vi "Write_Single_Impedance_Meas.vi"(0 "Meta-Data Array":dbl[](array[numeric])=[1.0], 3 "Mean Signal\nImpedance cluster":T3, 4 "Current":waveform(dbl)[](array[waveform]), 5 "Run Impedances array":dbl[][](array[numeric]), 6 "Voltage":waveform(dbl)[](array[waveform]), 7 "Compensation and Gain":T1={"Rg_Vmon"=5000.0, "Rg_Imon"=5000.0, "ESL_Cal"=2.5e-07, "ESR_Cal"=0.0, "Cp_Cal"=0.0, "Rp_Cal"=0.0, "Use Open/Short\nCompensation"=FALSE, "R_Shunt"=10000.0, "RLoad"=1000000000.0, "RLoad_Meas"=1000000000.0} {"RLoad_Meas" format="%#_6p"; "RLoad" format="%#_6p"}, 8 "Test Params Cluster":T2={"Test Freq. (Hz)"=0.0, "Output Signal Amplitude\nVolts Pk"=0.0, "Sampling Time (s)"=0.0, "Sampling Rate (Hz)"=0.0, "Output Channel"="Dev2/ao0", "Current Channel"="Dev2/ai0", "Voltage Channel"="Dev2/ai0", "Trigger Channel"="/Dev2/ao/StartTrigger", "Number of runs"=5}, 9 "Experiment Title":string="Experiment Title", 10 "File Name String":string="Test", 11 "Path":path=path "C:/Users/MPI/Documents/Test Saving Data") -> ()   [LabVIEW 2022 SP3]
panel:
  out "TDMS path":path=path "C:/Users/MPI/Documents/Test Saving Data/2022_01_06_23_07_06_Test.tdms"
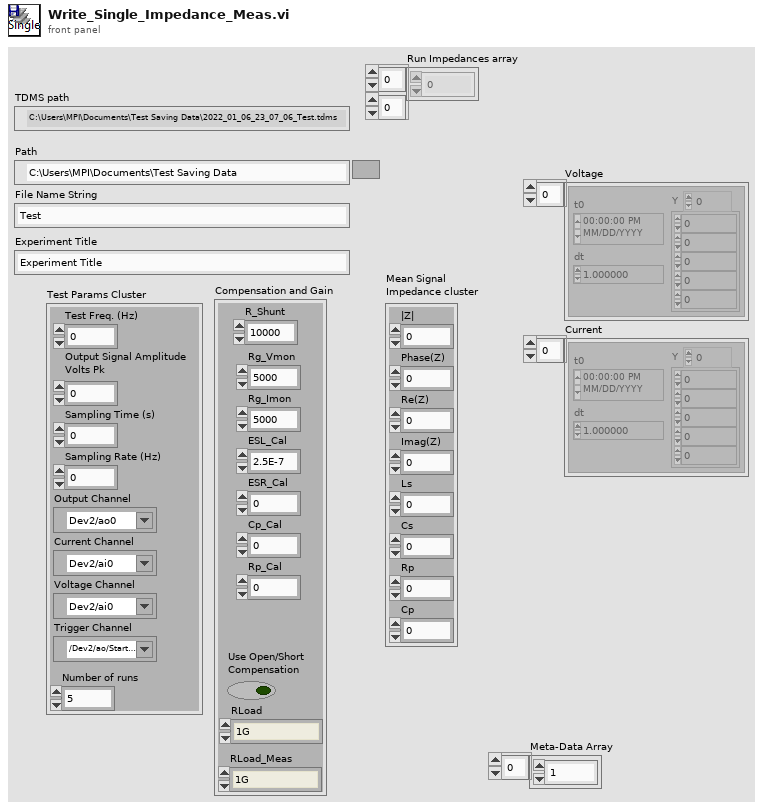
[diagram p1: front panel]
types:
  T1 = cluster{"Rg_Vmon":dbl, "Rg_Imon":dbl, "ESL_Cal":dbl, "ESR_Cal":dbl, "Cp_Cal":dbl, "Rp_Cal":dbl, "Use Open/Short\nCompensation":bool, "R_Shunt":dbl, "RLoad":dbl, "RLoad_Meas":dbl}
  T2 = cluster{"Test Freq. (Hz)":dbl, "Output Signal Amplitude\nVolts Pk":dbl, "Sampling Time (s)":dbl, "Sampling Rate (Hz)":dbl, "Output Channel":tag, "Current Channel":tag, "Voltage Channel":tag, "Trigger Channel":tag, "Number of runs":i32}
  T3 = cluster{"|Z|":dbl, "Phase(Z)":dbl, "Re(Z)":dbl, "Imag(Z)":dbl, "Ls":dbl, "Cs":dbl, "Rp":dbl, "Cp":dbl}
  T4 = enum16{"open", "open or create", "create or replace", "create", "open (read-only)"}
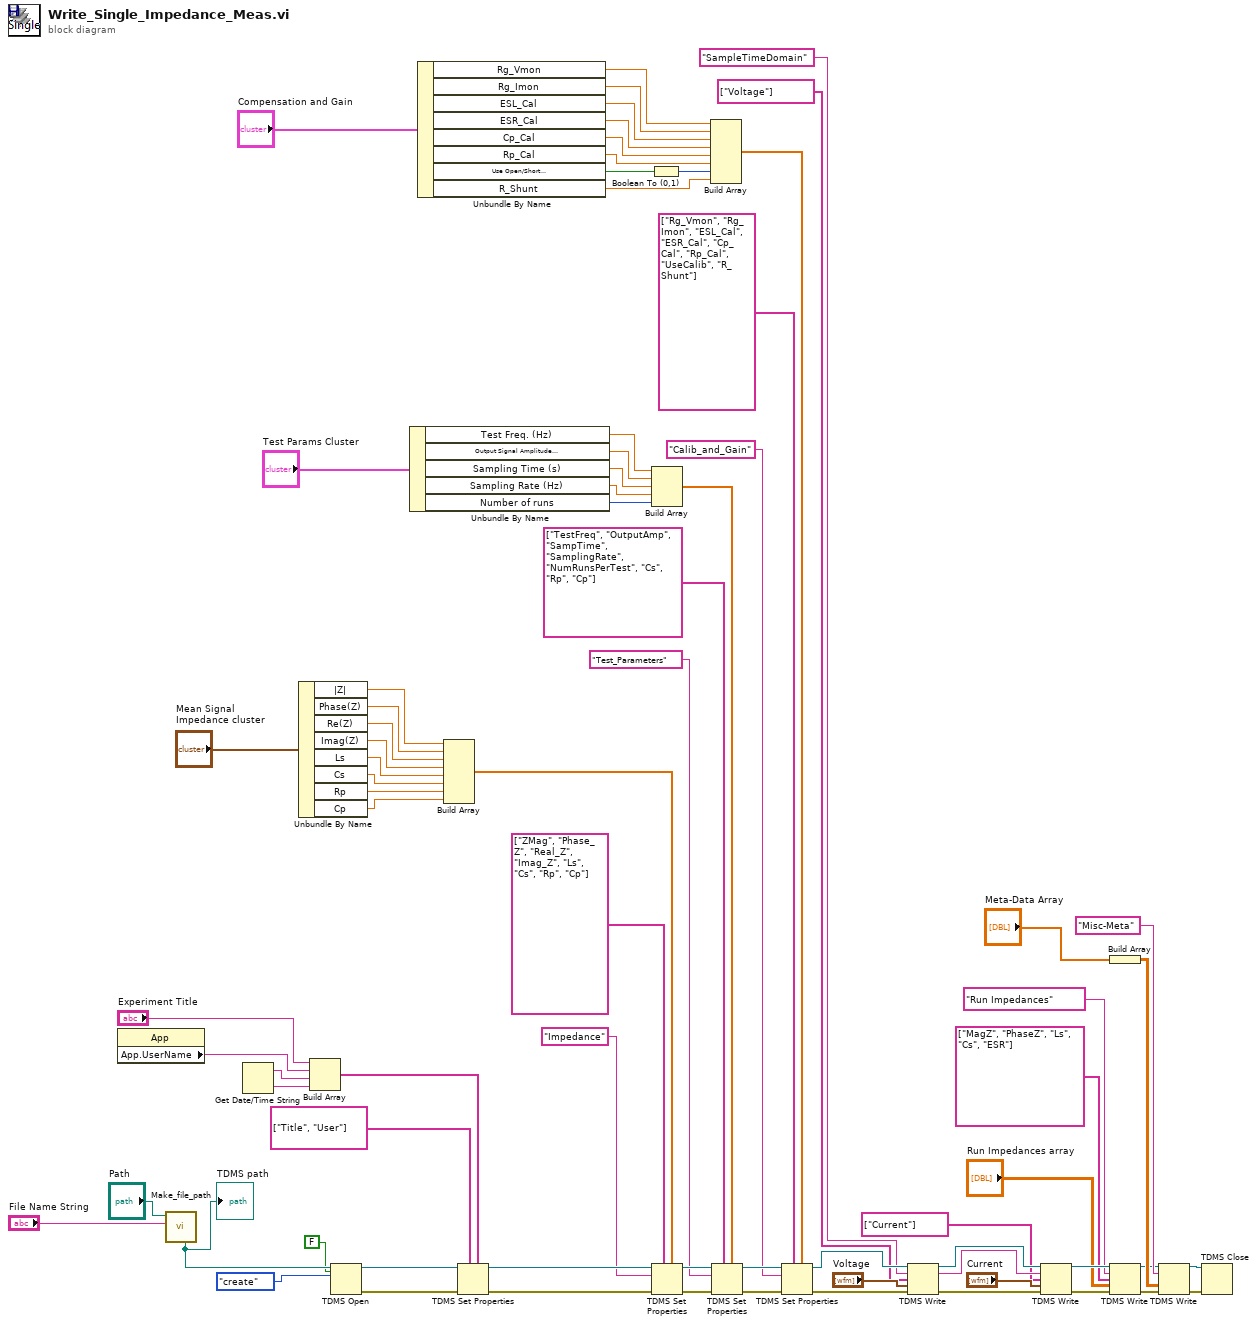
[diagram p0: block diagram]
diagram:
  n1 = property class="App"() -> ("App.UserName"=w69:string)  [unwired: 2 in, 2 out]
  n2 = call "Make_file_path.vi"("File Name String"="File Name String", "Base path"="Path") -> ("TDMS path"=w75:path)  [unwired: 9 in]
  "TDMS path" <- w75
  n3 = Get Date/Time String() -> (date string=w53:string, time string=w52:string)  [unwired: 3 in]
  n4 = Unbundle By Name("Mean Signal\nImpedance cluster") -> ("|Z|"=w62:dbl, "Phase(Z)"=w60:dbl, "Re(Z)"=w59:dbl, "Imag(Z)"=w58:dbl, "Ls"=w57:dbl, "Cs"=w56:dbl, "Rp"=w55:dbl, "Cp"=w54:dbl)
  n5 = Build Array("Experiment Title", w69, w53, w52) -> (w68:string[])
  n6 = TDMS Open(5:FALSE ("create index file? (T)"), 10:T4."create" ("operation (0:open)"), 11:w75) -> (0:w50:errorcluster, 3:w66:refnum<k34>)  [unwired: 4 in]
  n7 = Unbundle By Name("Test Params Cluster") -> ("Test Freq. (Hz)"=w41:dbl, "Output Signal Amplitude\nVolts Pk"=w42:dbl, "Sampling Time (s)"=w43:dbl, "Sampling Rate (Hz)"=w44:dbl, "Number of runs"=w8:i32)
  n8 = Unbundle By Name("Compensation and Gain") -> ("Rg_Vmon"=w33:dbl, "Rg_Imon"=w32:dbl, "ESL_Cal"=w31:dbl, "ESR_Cal"=w30:dbl, "Cp_Cal"=w29:dbl, "Rp_Cal"=w28:dbl, "Use Open/Short\nCompensation"=w27:bool, "R_Shunt"=w24:dbl)
  n9 = Build Array(w62, w60, w59, w58, w57, w56, w55, w54) -> (w63:dbl[])
  n10 = TDMS Set Properties(5:w68, 7:string[] ["Title", "User"] ("property names"), 8:w50, 11:w66) -> (0:w51:errorcluster, 3:w65:refnum<k34>)  [unwired: 4 out]
  n11 = Boolean To (0,1)(Boolean=w27) -> (0, 1=w26:i16)
  n12 = Build Array(w41, w42, w43, w44, w8) -> (w40:dbl[])
  n13 = TDMS Set Properties(5:w63, 7:string[] ["ZMag", "Phase_Z", "Real_Z", "Imag_Z", "Ls", "Cs", "Rp", "Cp"] ("property names"), 8:w51, 10:"Impedance" ("group name"), 11:w65) -> (0:w46:errorcluster, 3:w47:refnum<k34>)  [unwired: 3 out]
  n14 = Build Array(w33, w32, w31, w30, w29, w28, w26, w24) -> (w25:dbl[])
  n15 = TDMS Set Properties(5:w40, 7:string[] ["TestFreq", "OutputAmp", "SampTime", "SamplingRate", "NumRunsPerTest", "Cs", "Rp", "Cp"] ("property names"), 8:w46, 10:"Test_Parameters" ("group name"), 11:w47) -> (0:w36:errorcluster, 3:w37:refnum<k34>)  [unwired: 3 out]
  n16 = TDMS Set Properties(5:w25, 7:string[] ["Rg_Vmon", "Rg_Imon", "ESL_Cal", "ESR_Cal", "Cp_Cal", "Rp_Cal", "UseCalib", "R_Shunt"] ("property names"), 8:w36, 10:"Calib_and_Gain" ("group name"), 11:w37) -> (0:w20:errorcluster, 3:w23:refnum<k34>)  [unwired: 3 out]
  n17 = TDMS Write(0:w23, 5:"SampleTimeDomain" ("group name in (Untitled)"), 7:string[] ["Voltage"] ("channel name(s) in (Untitled)"), 9:"Voltage", 11:w20) -> (4:w22:refnum<k34>, 6:w16:string, 15:w21:errorcluster)  [unwired: 1 in, 1 out]
  n18 = TDMS Write(0:w22, 5:w16, 7:string[] ["Current"] ("channel name(s) in (Untitled)"), 9:"Current", 11:w21) -> (4:w12:refnum<k34>, 15:w13:errorcluster)  [unwired: 1 in, 2 out]
  n19 = Build Array("Meta-Data Array") -> (w5:dbl[][])
  n20 = TDMS Write(0:w12, 5:"Run Impedances" ("group name in (Untitled)"), 7:string[] ["MagZ", "PhaseZ", "Ls", "Cs", "ESR"] ("channel name(s) in (Untitled)"), 9:"Run Impedances array", 11:w13) -> (4:w4:refnum<k34>, 15:w1:errorcluster)  [unwired: 1 in, 2 out]
  n21 = TDMS Write(0:w4, 5:"Misc-Meta" ("group name in (Untitled)"), 9:w5, 11:w1) -> (4:w3:refnum<k34>, 15:w2:errorcluster)  [unwired: 2 in, 2 out]
  n22 = TDMS Close(8:w2, 11:w3) -> ()  [unwired: 2 out]
